vi "Format Data for Unicode-Export.vi"(7 "LT.Data.Languages":cluster{"ANSI":string[], "Unicode":string[]}, 11 "Translations":T1[](array[typedef])) -> (3 "string":string)   [LabVIEW 2019, in "Language Editor.lvlib"]
doc: "- - -\nCopyright (c) 2026, Merecs Engineering GmbH"
uses:
  Language Editor.lvlib
  Language Selection/TypeDefs/Cluster Language.ctl
  Language Selection/TypeDefs/Cluster PropertyTranslation.ctl
  Language Selection/TypeDefs/Enum Property Type.ctl
  <vilib>/addons/Tools/Unicode/_subVIs/Convert ASCII to UTF-16LE (Scalar).vi
  <vilib>/addons/Tools/Unicode/_subVIs/Convert ASCII to UTF-16LE (1D).vi
  <vilib>/addons/Tools/Unicode/UI Unicode Tools.lvlib
  Language Selection/Language Selection.lvlib
panel:
  # "Connector Pane"
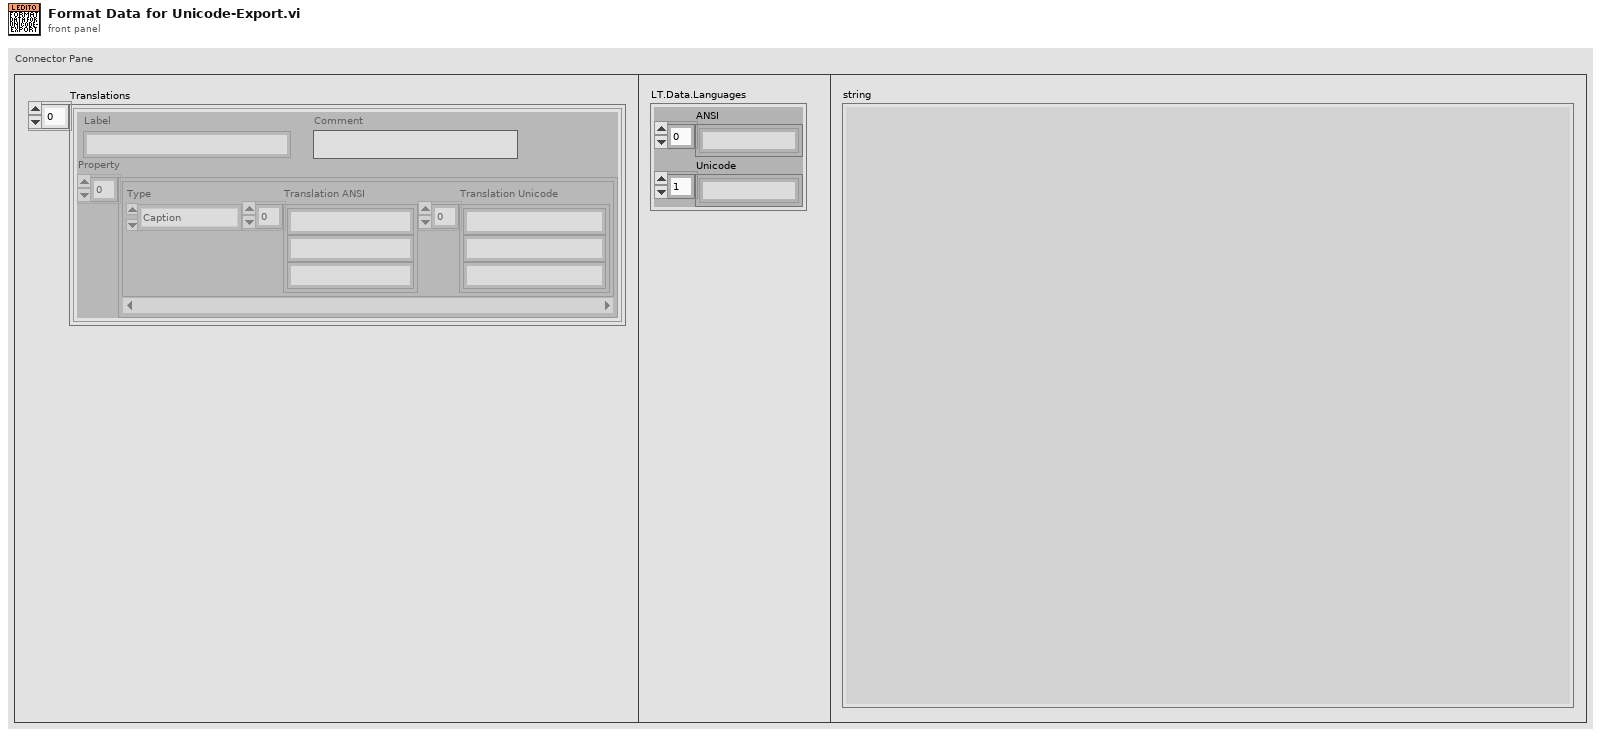
[diagram p1: front panel]
types:
  T1 = typedef "Language Selection.lvlib/Cluster Language.ctl" = cluster{"Label":string, "Comment":string, "Property":T2[]}
  T2 = typedef "Language Selection.lvlib/Cluster PropertyTranslation.ctl" = cluster{"Type":T3, "Translation ANSI":string[], "Translation Unicode":string[]}
  T3 = typedef "Language Selection.lvlib/Enum Property Type.ctl" = enum16{"NA", "Caption", "String Value", "Boolean Text", "Ring Strings", "1D Array Elements", "2D Array Elements", "(MC)Listbox Header", "(MC)Listbox Items", "Tab Pages Names", "X & Y GraphChart", "Plot Names", "Table Headers", "Table Items", "TipStrip", "Combobox Strings", "Cursor Name", "Tree Col Headers"}
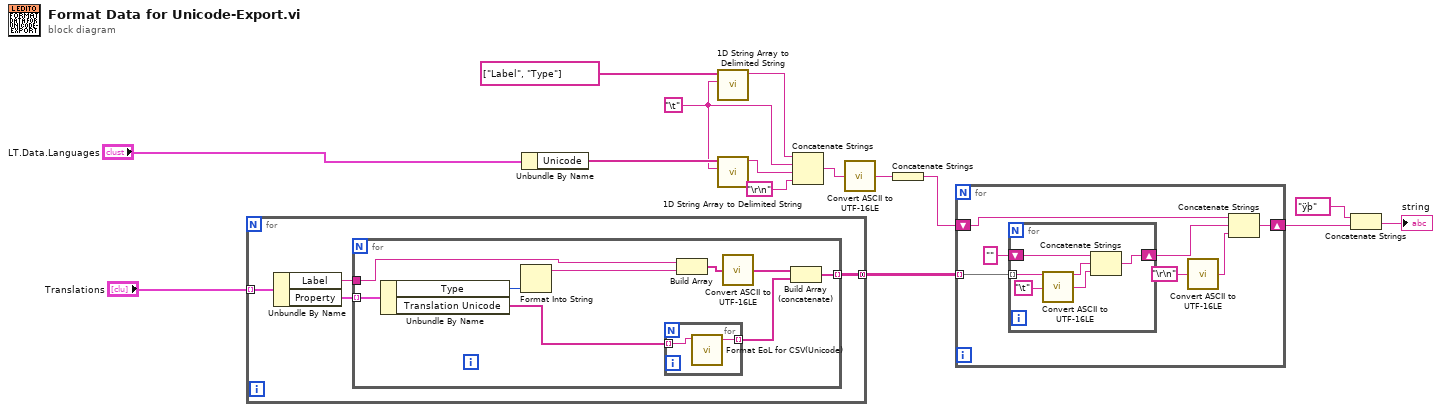
[diagram p0: block diagram]
diagram:
  w10 = "\t"
  n1 = for {
    tunnel: "Translations" -> [w19] mode=indexing
    tunnel: [w16] -> w9 mode=concatenating
    n2 = Unbundle By Name(w19) -> ("Label"=w17:string, "Property"=w18:T2[])
    n3 = for {
      tunnel: w18 -> [w28] mode=indexing
      tunnel: w17 -> [w24]
      tunnel: [w23] -> w16 mode=indexing
      n4 = Unbundle By Name(w28) -> ("Type"=w27:T3, "Translation Unicode"=w21:string[])
      n5 = Format Into String(w27) -> (resulting string=w25:string)  [unwired: 3 in, 1 out]
      n6 = for {
        tunnel: w21 -> [w30] mode=indexing
        tunnel: [w29] -> w20 mode=indexing
        n7 = call "Format EoL for CSV(Unicode).vi"("base string"=w30) -> ("String out"=w29:string)  [unwired: 10 in]
      }
      n8 = Build Array(w24, w25) -> (w26:string[])
      n9 = call-poly <vilib>:"Convert ASCII to UTF-16LE.vi"("ASCII"=w26) -> ("Unicode"=w22:string[])  [unwired: 4 in]
      n10 = Build Array (concatenate)(w22, w20) -> (w23:string[])
    }
  }
  n11 = Unbundle By Name("LT.Data.Languages") -> ("Unicode"=w13:string[])
  n12 = call <vilib>:"1D String Array to Delimited String.vi"("delimiter"=w10, "string array"=string[] ["Label", "Type"] ("new element/subarray")) -> ("delimited string"=w12:string)  [unwired: 9 in]
  n13 = call <vilib>:"1D String Array to Delimited String.vi"("delimiter"=w10, "string array"=w13) -> ("delimited string"=w11:string)  [unwired: 9 in]
  n14 = Concatenate Strings(w12, w10, w11, "\r\n") -> (w8:string)
  n15 = call-poly <vilib>:"Convert ASCII to UTF-16LE.vi"("ASCII"=w8) -> ("Unicode"=w4:string)  [unwired: 4 in]
  n16 = Concatenate Strings(w4) -> (w3:string)
  n17 = for {
    tunnel: w9 -> [w37] mode=indexing
    shift-right: [w34] -> w5
    shift-left: w3 -> [w35]
    n18 = for {
      shift-right: [w40] -> w36
      shift-left: "" ("string") -> [w42]
      tunnel: w37 -> [w41] mode=indexing
      n19 = call-poly <vilib>:"Convert ASCII to UTF-16LE.vi"("ASCII"="\t") -> ("Unicode"=w39:string)  [unwired: 4 in]
      n20 = Concatenate Strings(w42, w41, w39) -> (w40:string)
    }
    n21 = call-poly <vilib>:"Convert ASCII to UTF-16LE.vi"("ASCII"="\r\n") -> ("Unicode"=w31:string)  [unwired: 4 in]
    n22 = Concatenate Strings(w35, w36, w31) -> (w34:string)
  }
  n23 = Concatenate Strings("ÿþ" ("string"), w5) -> (→"string":string)
